vi "RemoteVI Fixture.vi"() -> ()   [LabVIEW 2020]
doc: "Event-logging test fixture of the RemoteVI integration tests (tests\\lv). At start it truncates or creates the log file (Log Path, or RemoteVI Fixture.log in the system temp directory when Log Path is empty), writes one layout line per logged control with its body rectangle in panel-image coordinates, publishes its own front panel with RemoteVI Start.vi on port 8089 and writes ready. An event loop then appends one tab-separated line per handled event - value changes of Switch, Button, Number, Text, Mode and Tab (Tab registered dynamically, because the tab control is pasted in after generation), mouse down and up on Switch, Button, Number and Text, mouse enter and leave on Button, key down on Text and Number, double click on List with the row, mouse wheel on Number with the delta, the selection in the run-time shortcut menu of Text by item tag (the menu is rebuilt in Shortcut Menu Activation? as Top and More with the submenu item Deep), the selection in the VI's run-time menu bar by item tag (built at start: one menu Fixture with Say Hello (tag Hello) and the submenu More with Deep Bar (tag DeepBar)), the answer of the Two Button Dialog Proceed? (Yes / No) that the latched button Ask opens (dialog TRUE or FALSE) and the result of the native File Dialog that the latched button Open opens (file and the path, or CANCELLED) - in the format documented in tests\\lv\\harness.mjs, while a parallel loop redraws a moving sine on Graph every 50 ms and logs scroll x y whenever the panel was scrolled (Front Panel Window:Origin changed); 1.5 s after the last scroll it scrolls the panel back to 0,0, so a later test run finds the controls where the layout lines say. Stop ends both loops, the log is closed and RemoteVI Stop.vi releases the port. error out merges every error path."
uses:
  source/RemoteVI.lvlib
panel:
  in  "Tab":enum32{"One", "Two"}(tab)
  out "error out":errorcluster
  out "Graph":dbl[](graph)
  in  "Stop":bool
  in  "Open":bool
  in  "Ask":bool
  in  "List":i32(listbox)
  in  "Mode":i32(ring) items=["Off", "Slow", "Fast"]
  in  "Text":string
  in  "Number":dbl
  in  "Button":bool
  in  "Switch":bool
  in  "Log Path":path
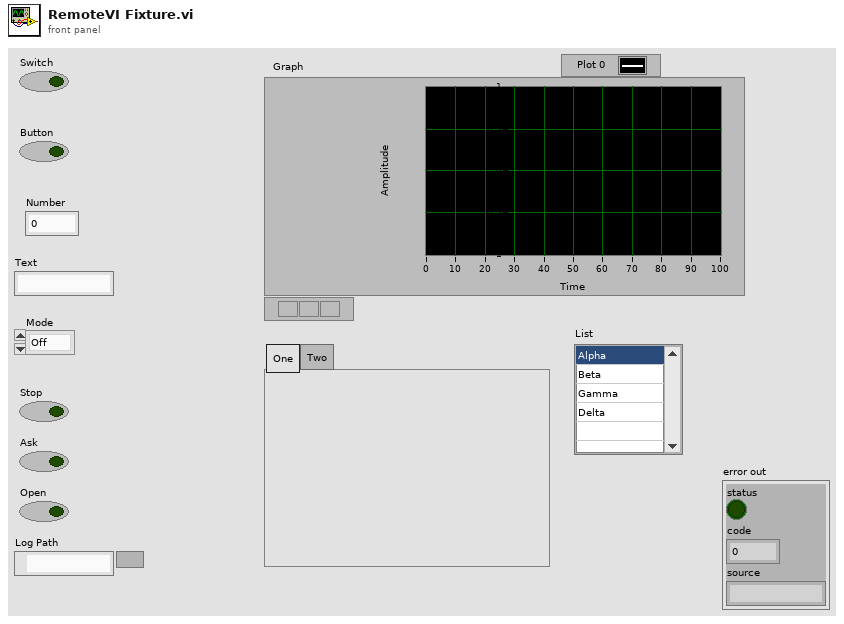
[diagram p1: front panel]
types:
  T1 = enum16{"open", "replace", "create", "open or create", "replace or create", "replace or create with confirmation"}
  T2 = typedef "LVPointTypeDef.ctl" = cluster{"Horizontal":i16, "Vertical":i16}
  T3 = typedef "LVPoint32TypeDef.ctl" = cluster{"Horizontal":i32, "Vertical":i32}
  T4 = cluster{"Shift":bool, "Ctrl":bool, "Alt":bool, "Cmd":bool, "Opt":bool}
  T5 = typedef "eventvkey.ctl" = enum16{"ASCII", "Enter", "Return", "Shift", "Ctrl", "Alt", "Cmd", "Opt", "Caps", "NumLock", "Clear", "Break", "Up", "Down", "Left", "Right", "Insert", "Delete", "Home", "End", "PageUp", "PageDown", "Escape", "Help", "Pause", "ScrollLock", "F1", "F2", "F3", "F4", "F5", "F6", "F7", "F8", "F9", "F10", "F11", "F12", "F13", "F14", "F15", "F16", "F17", "F18", "F19", "F20", "F21", "F22", "F23", "F24", "Play", "VolumeUp", "VolumeDown", "Mute", "Two Byte Char"}
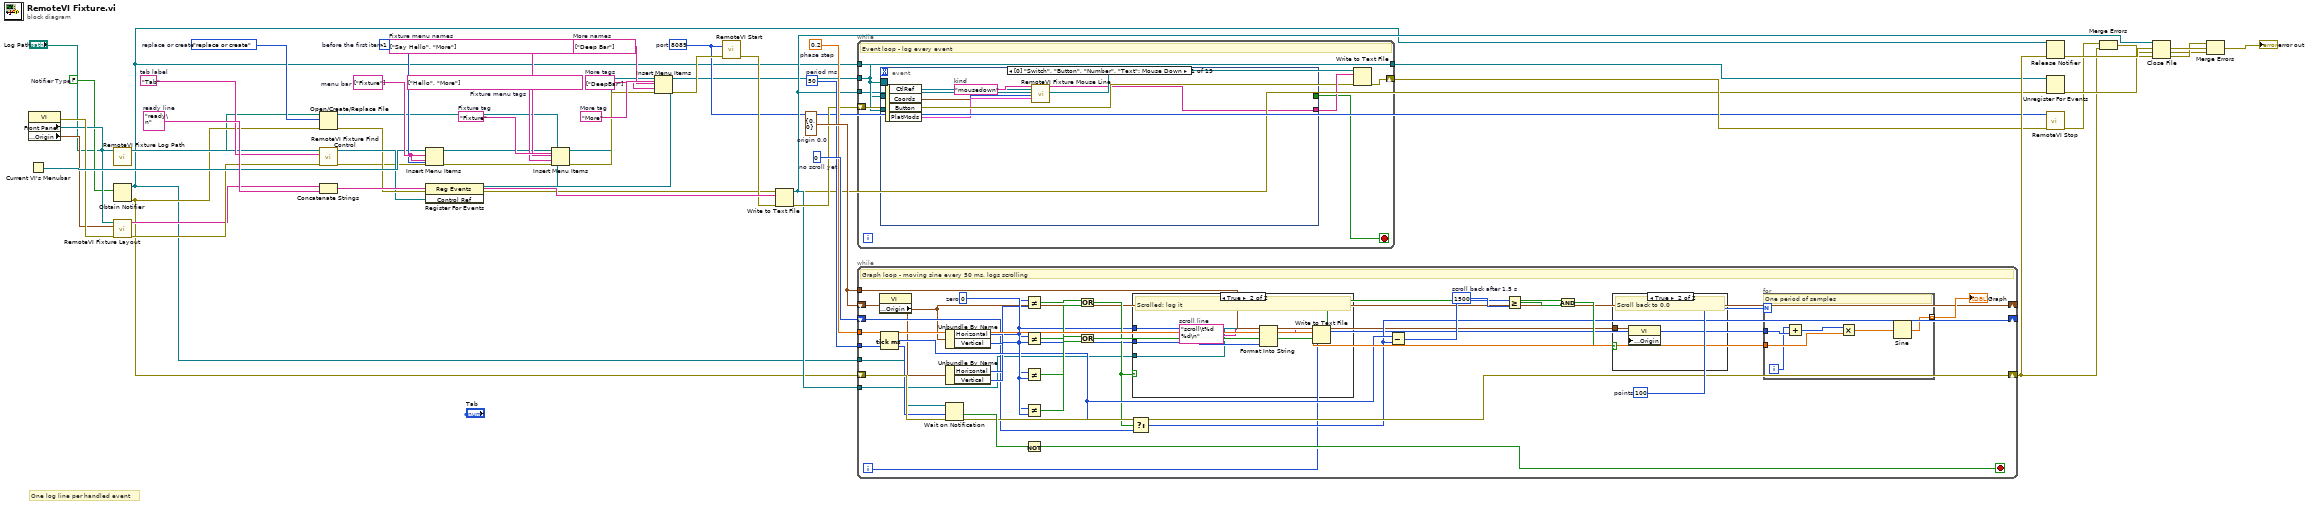
[diagram p0: block diagram]
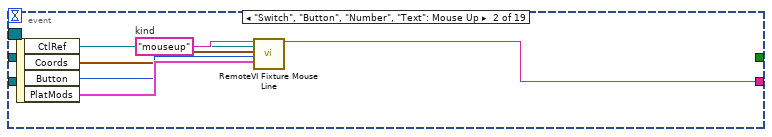
[diagram p4: hidden frame]
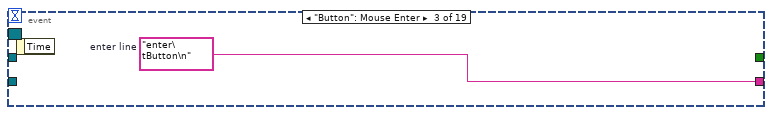
[diagram p5: hidden frame]
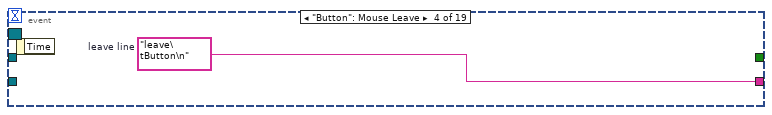
[diagram p6: hidden frame]
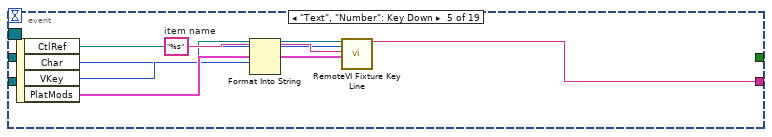
[diagram p7: hidden frame]
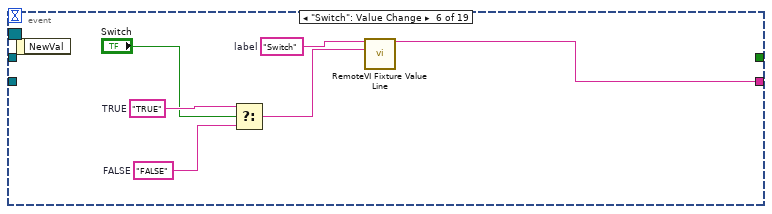
[diagram p8: hidden frame]
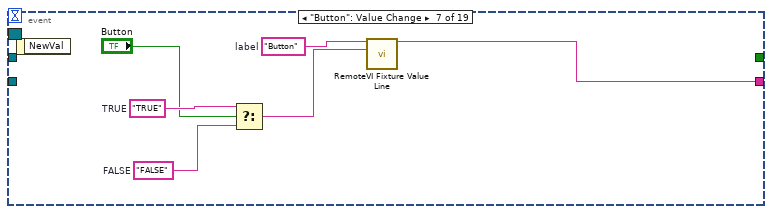
[diagram p9: hidden frame]
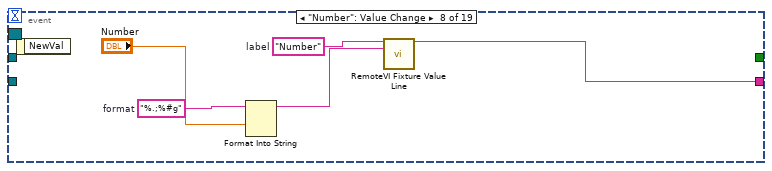
[diagram p10: hidden frame]
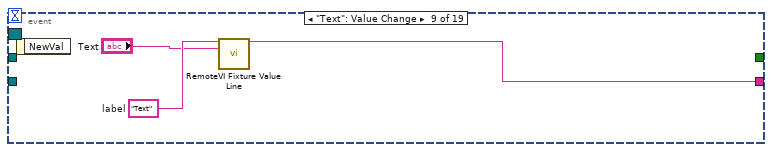
[diagram p11: hidden frame]
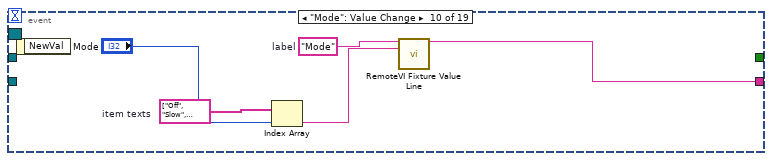
[diagram p12: hidden frame]
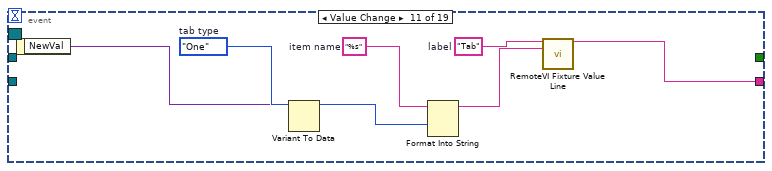
[diagram p13: hidden frame]
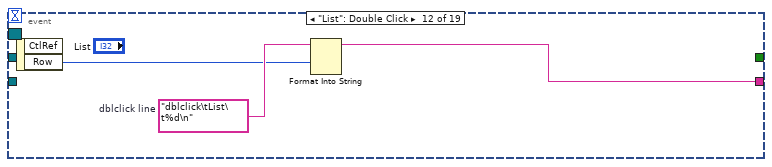
[diagram p14: hidden frame]
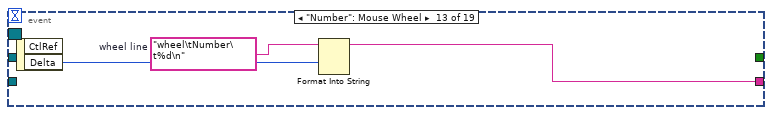
[diagram p15: hidden frame]
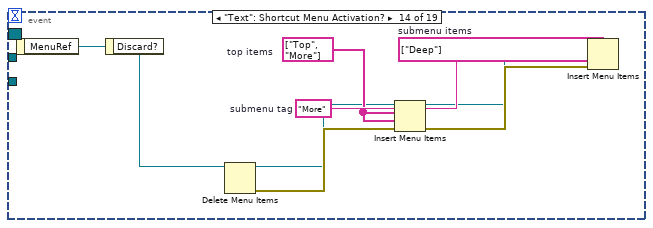
[diagram p16: hidden frame]
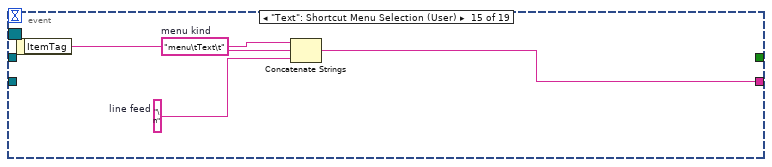
[diagram p17: hidden frame]
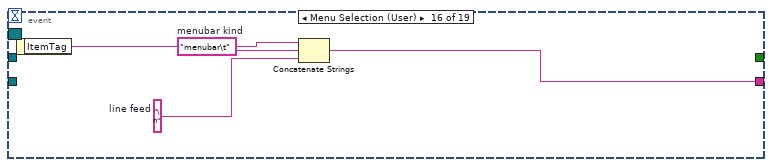
[diagram p18: hidden frame]
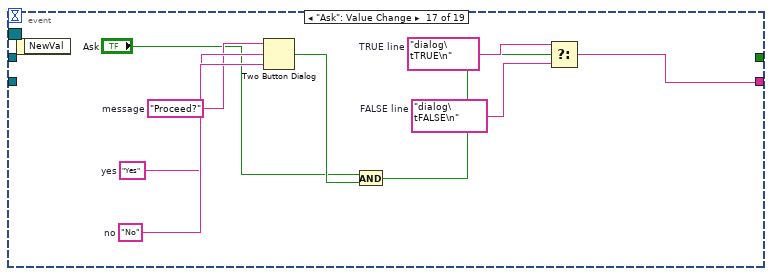
[diagram p19: hidden frame]
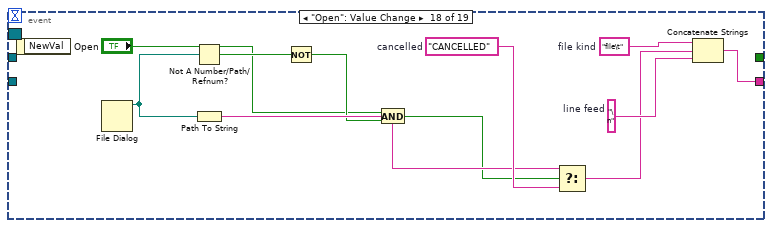
[diagram p20: hidden frame]
diagram:
  w44 = u32 0  # no scroll yet
  w43 = cluster{"Horizontal":i32, "Vertical":i32} {"Horizontal"=0, "Vertical"=0}  # origin 0,0
  w42 = 50  # period ms
  w41 = 0.2  # phase step
  w35 = "ready\n"  # ready line
  w32 = "More"  # More tag
  w31 = string[] ["DeepBar"]  # More tags
  w30 = string[] ["Deep Bar"]  # More names
  w27 = "Fixture"  # Fixture tag
  w26 = string[] ["Hello", "More"]  # Fixture menu tags
  w25 = string[] ["Say Hello", "More"]  # Fixture menu names
  w22 = string[] ["Fixture"]  # menu bar
  w21 = -1  # before the first item
  w19 = u16 8089  # port
  w14 = "Tab"  # tab label
  w6 = T1."replace or create"  # replace or create
  w3 = FALSE  # Notifier Type
  # "One log line per handled event"
  n1 = property class="VI"() -> (error out=w11:errorcluster, "Front Panel"=w9:refnum<vi>, "Front Panel Window:Origin"=w10:T2)  [unwired: 2 in, 1 out]
  n2 = Current VI's Menubar() -> (w20:refnum<k9>)
  n3 = call "RemoteVI Fixture Log Path.vi"("Log Path"="Log Path") -> ("path"=w2:path)  [unwired: 13 in, 1 out]
  n4 = Obtain Notifier(notification data type=w3) -> (notifier out=w4:refnum<notifier>, error out=w5:errorcluster)  [unwired: 3 in, 1 out]
  n5 = call "RemoteVI Fixture Layout.vi"("Panel"=w9, "Origin"=w10, "error in"=w11) -> ("layout"=w12:string, "error out"=w13:errorcluster)  [unwired: 11 in]
  n6 = Open/Create/Replace File(file path (use dialog)=w2, error in=w5, operation (0:open)=w6) -> (refnum out=w7:refnum<file>, error out=w8:errorcluster)  [unwired: 3 in, 1 out]
  n7 = call "RemoteVI Fixture Find Control.vi"("Panel"=w9, "label"=w14, "error in"=w13) -> ("Control Ref"=w15:refnum<vi>, "error out"=w16:errorcluster)  [unwired: 11 in]
  n8 = Concatenate Strings(w12, w35) -> (w36:string)
  n9 = Insert Menu Items(4:w21, 6:w8, 7:w22, 8:w22, 9:w20) -> (0:w24:errorcluster, 3:w23:refnum<k9>)  [unwired: 1 in, 1 out]
  n10 = register-events(error in=w16, w15) -> (reference out=w17:refnum<event-registration>, error out=w18:errorcluster)  [unwired: 1 in]
  n11 = Insert Menu Items(5:w27, 6:w24, 7:w26, 8:w25, 9:w23) -> (0:w29:errorcluster, 3:w28:refnum<k9>)  [unwired: 1 in, 1 out]
  n12 = Insert Menu Items(5:w32, 6:w29, 7:w31, 8:w30, 9:w28) -> (0:w33:errorcluster)  [unwired: 1 in, 2 out]
  n13 = call "RemoteVI Start.vi"("port"=w19, "error in"=w33) -> ("error out"=w34:errorcluster)  [unwired: 12 in, 1 out]
  n14 = Write to Text File(file (use dialog)=w7, text=w36, error in=w34) -> (refnum out=w37:refnum<file>, error out=w38:errorcluster)  [unwired: 1 in, 1 out]
  n15 = while {
    tunnel: w4 -> [w52]
    tunnel: w17 -> [w54]
    tunnel: [w54] -> w40
    tunnel: w37 -> [w53]
    shift-right: [w56] -> w39
    shift-left: w38 -> [w55]
    stop <- w57 stop-if-true
    # "Event loop - log every event"
    n16 = event shown="[0] \"Switch\", \"Button\", \"Number\", \"Text\": Mouse Down" {
      selector: w54 -> [_ _ _ _ _ _ _ _ _ _ _ _ _ _ _ _ _ _ _]
      dyn-events: _ -> [_ _ _ _ _ _ _ _ _ _ _ _ _ _ _ _ _ _ _]
      timeout: _ -> [_ _ _ _ _ _ _ _ _ _ _ _ _ _ _ _ _ _ _]
      tunnel: [_ _ _ _ _ _ _ _ _ _ _ _ _ _ _ _ _ _ "Stop"] -> w57
      tunnel: w52 -> [_ _ _ _ _ _ _ _ _ _ _ _ _ _ _ _ _ _ w154]
      tunnel: [w64 w70 w71 w72 w79 w85 w91 w96 w99 w104 w111 w114 w117 _ w129 w133 w142 w153 _] -> w58
      tunnel: w54 -> [_ _ _ _ _ _ _ _ _ _ _ _ _ _ _ _ _ _ _]
      event "Switch", "Button", "Number", "Text": Mouse Down {
        w63 = "mousedown"  # kind
        n17 = event-data() -> ("CtlRef"=w59:refnum<vi>, "Coords"=w60:T3, "Button"=w61:u16, "PlatMods"=w62:T4)  [unwired: 1 in]
        n18 = call "RemoteVI Fixture Mouse Line.vi"("kind"=w63, "CtlRef"=w59, "Coords"=w60, "Button"=w61, "PlatMods"=w62) -> ("line"=w64:string)  [unwired: 13 in, 1 out]
      }
      event "Switch", "Button", "Number", "Text": Mouse Up {
        w69 = "mouseup"  # kind
        n19 = event-data() -> ("CtlRef"=w65:refnum<vi>, "Coords"=w66:T3, "Button"=w67:u16, "PlatMods"=w68:T4)  [unwired: 1 in]
        n20 = call "RemoteVI Fixture Mouse Line.vi"("kind"=w69, "CtlRef"=w65, "Coords"=w66, "Button"=w67, "PlatMods"=w68) -> ("line"=w70:string)  [unwired: 13 in, 1 out]
      }
      event "Button": Mouse Enter {
        w71 = "enter\tButton\n"  # enter line
        n21 = event-data() -> ()  [unwired: 1 in, 1 out]
      }
      event "Button": Mouse Leave {
        w72 = "leave\tButton\n"  # leave line
        n22 = event-data() -> ()  [unwired: 1 in, 1 out]
      }
      event "Text", "Number": Key Down {
        w77 = "%s"  # item name
        n23 = event-data() -> ("CtlRef"=w73:refnum<vi>, "Char"=w74:i16, "VKey"=w75:T5, "PlatMods"=w76:T4)  [unwired: 1 in]
        n24 = Format Into String(format string=w77, w75) -> (resulting string=w78:string)  [unwired: 2 in, 1 out]
        n25 = call "RemoteVI Fixture Key Line.vi"("CtlRef"=w73, "Char"=w74, "VKey"=w78, "PlatMods"=w76) -> ("line"=w79:string)  [unwired: 14 in, 1 out]
      }
      event "Switch": Value Change {
        w83 = "FALSE"  # FALSE
        w82 = "TRUE"  # TRUE
        w81 = "Switch"  # label
        n26 = event-data() -> ()  [unwired: 1 in, 1 out]
        n27 = Select(t=w82, s="Switch", f=w83) -> (s? t:f=w84:string)
        n28 = call "RemoteVI Fixture Value Line.vi"("label"=w81, "value"=w84) -> ("line"=w85:string)  [unwired: 12 in, 1 out]
      }
      event "Button": Value Change {
        w89 = "FALSE"  # FALSE
        w88 = "TRUE"  # TRUE
        w87 = "Button"  # label
        n29 = event-data() -> ()  [unwired: 1 in, 1 out]
        n30 = Select(t=w88, s="Button", f=w89) -> (s? t:f=w90:string)
        n31 = call "RemoteVI Fixture Value Line.vi"("label"=w87, "value"=w90) -> ("line"=w91:string)  [unwired: 12 in, 1 out]
      }
      event "Number": Value Change {
        w94 = "%.;%#g"  # format
        w93 = "Number"  # label
        n32 = event-data() -> ()  [unwired: 1 in, 1 out]
        n33 = Format Into String(format string=w94, "Number") -> (resulting string=w95:string)  [unwired: 2 in, 1 out]
        n34 = call "RemoteVI Fixture Value Line.vi"("label"=w93, "value"=w95) -> ("line"=w96:string)  [unwired: 12 in, 1 out]
      }
      event "Text": Value Change {
        w98 = "Text"  # label
        n35 = event-data() -> ()  [unwired: 1 in, 1 out]
        n36 = call "RemoteVI Fixture Value Line.vi"("label"=w98, "value"="Text") -> ("line"=w99:string)  [unwired: 12 in, 1 out]
      }
      event "Mode": Value Change {
        w102 = string[] ["Off", "Slow", "Fast"]  # item texts
        w101 = "Mode"  # label
        n37 = event-data() -> ()  [unwired: 1 in, 1 out]
        n38 = Index Array(array=w102, index="Mode") -> (element=w103:string)
        n39 = call "RemoteVI Fixture Value Line.vi"("label"=w101, "value"=w103) -> ("line"=w104:string)  [unwired: 12 in, 1 out]
      }
      event Value Change {
        w109 = "%s"  # item name
        w108 = "Tab"  # label
        w106 = enum32{"One", "Two"}."One"  # tab type
        n40 = event-data() -> ("NewVal"=w105:variant)  [unwired: 1 in]
        n41 = Variant To Data(type=w106, Variant=w105) -> (data=w107:enum32{"One", "Two"})  [unwired: 1 in, 1 out]
        n42 = Format Into String(format string=w109, w107) -> (resulting string=w110:string)  [unwired: 2 in, 1 out]
        n43 = call "RemoteVI Fixture Value Line.vi"("label"=w108, "value"=w110) -> ("line"=w111:string)  [unwired: 12 in, 1 out]
      }
      event "List": Double Click {
        w113 = "dblclick\tList\t%d\n"  # dblclick line
        n44 = event-data() -> ("Row"=w112:i32)  [unwired: 1 in, 1 out]
        n45 = Format Into String(format string=w113, w112) -> (resulting string=w114:string)  [unwired: 2 in, 1 out]
      }
      event "Number": Mouse Wheel {
        w116 = "wheel\tNumber\t%d\n"  # wheel line
        n46 = event-data() -> ("Delta"=w115:i32)  [unwired: 1 in, 1 out]
        n47 = Format Into String(format string=w116, w115) -> (resulting string=w117:string)  [unwired: 2 in, 1 out]
      }
      event "Text": Shortcut Menu Activation? {
        w125 = "More"  # submenu tag
        w124 = string[] ["Deep"]  # submenu items
        w121 = string[] ["Top", "More"]  # top items
        n48 = event-data() -> ("MenuRef"=w118:refnum<k9>)  [unwired: 1 in]
        n49 = event-data() -> ()  [unwired: 2 in, 1 out]
        n50 = Delete Menu Items(9:w118) -> (0:w120:errorcluster, 3:w119:refnum<k9>)  [unwired: 3 in]
        n51 = Insert Menu Items(6:w120, 7:w121, 8:w121, 9:w119) -> (0:w123:errorcluster, 3:w122:refnum<k9>)  [unwired: 2 in, 1 out]
        n52 = Insert Menu Items(5:w125, 6:w123, 7:w124, 8:w124, 9:w122) -> ()  [unwired: 1 in, 3 out]
      }
      event "Text": Shortcut Menu Selection (User) {
        w128 = "\n"  # line feed
        w127 = "menu\tText\t"  # menu kind
        n53 = event-data() -> ("ItemTag"=w126:string)  [unwired: 1 in]
        n54 = Concatenate Strings(w127, w126, w128) -> (w129:string)
      }
      event Menu Selection (User) {
        w132 = "\n"  # line feed
        w131 = "menubar\t"  # menubar kind
        n55 = event-data() -> ("ItemTag"=w130:string)  [unwired: 1 in]
        n56 = Concatenate Strings(w131, w130, w132) -> (w133:string)
      }
      event "Ask": Value Change {
        w141 = "dialog\tFALSE\n"  # FALSE line
        w140 = "dialog\tTRUE\n"  # TRUE line
        w137 = "No"  # no
        w136 = "Yes"  # yes
        w135 = "Proceed?"  # message
        n57 = event-data() -> ()  [unwired: 1 in, 1 out]
        n58 = Two Button Dialog(message=w135, 1:w137, 2:w136) -> (T button?=w138:bool)
        n59 = And(x="Ask", y=w138) -> (x .and. y?=w139:bool)
        n60 = Select(t=w140, s=w139, f=w141) -> (s? t:f=w142:string)
      }
      event "Open": Value Change {
        w152 = "\n"  # line feed
        w151 = "file\t"  # file kind
        w149 = "CANCELLED"  # cancelled
        n61 = event-data() -> ()  [unwired: 1 in, 1 out]
        n62 = File Dialog() -> (3:w144:path)  [unwired: 7 in, 3 out]
        n63 = Not A Number/Path/Refnum?(number/path/refnum=w144) -> (NaN/Path/Refnum?=w145:bool)
        n64 = Path To String(path=w144) -> (string=w148:string)
        n65 = Not(x=w145) -> (.not. x?=w146:bool)
        n66 = And(x="Open", y=w146) -> (x .and. y?=w147:bool)
        n67 = Select(t=w148, s=w147, f=w149) -> (s? t:f=w150:string)
        n68 = Concatenate Strings(w151, w150, w152) -> (w153:string)
      }
      event "Stop": Value Change {
        n69 = event-data() -> ()  [unwired: 1 in, 1 out]
        n70 = Send Notification(notification="Stop", notifier=w154) -> ()  [unwired: 1 in, 2 out]
      }
    }
    n71 = Write to Text File(file (use dialog)=w53, text=w58, error in=w55) -> (error out=w56:errorcluster)  [unwired: 1 in, 2 out]
  }
  n72 = while {
    tunnel: w43 -> [w159]
    shift-right: [w161] -> _
    shift-left: w43 -> [w160]
    shift-right: [w163] -> _
    shift-left: w44 -> [w162]
    tunnel: w41 -> [w180]
    tunnel: w42 -> [w181]
    tunnel: w4 -> [w157]
    shift-right: [w183] -> w45
    shift-left: w5 -> [w182]
    tunnel: w37 -> [w158]
    i -> [w156]
    stop <- w187 stop-if-true
    w185 = 100  # points
    w177 = u32 1500  # scroll back after 1.5 s
    w172 = 0  # zero
    # "Graph loop - moving sine every 50 ms, logs scrolling"
    n73 = property class="VI"() -> ("Front Panel Window:Origin"=w161:T2)  [unwired: 2 in, 2 out]
    n74 = Tick Count (ms)() -> (millisecond timer value=w171:u32)
    n75 = Unbundle By Name(w161) -> ("Horizontal"=w164:i16, "Vertical"=w165:i16)
    n76 = Unbundle By Name(w160) -> ("Horizontal"=w166:i32, "Vertical"=w167:i32)
    n77 = Wait on Notification(notifier=w157, timeout in ms (-1)=w181, error in (no error)=w182) -> (timed out?=w184:bool, error out=w183:errorcluster)  [unwired: 1 in, 2 out]
    n78 = Not Equal?(x=w164, y=w166) -> (x != y?=w168:bool)
    n79 = Not Equal?(x=w165, y=w167) -> (x != y?=w169:bool)
    n80 = Not Equal?(x=w164, y=w172) -> (x != y?=w173:bool)
    n81 = Not Equal?(x=w165, y=w172) -> (x != y?=w174:bool)
    n82 = Not(x=w184) -> (.not. x?=w187:bool)
    n83 = Or(x=w168, y=w169) -> (x .or. y?=w170:bool)
    n84 = Or(x=w173, y=w174) -> (x .or. y?=w175:bool)
    n85 = case shown="True" w170 {
      tunnel: w164 -> [_ w196]
      tunnel: w165 -> [_ w197]
      tunnel: w158 -> [_ w195]
      frame False {
      }
      frame True {
        w198 = "scroll\t%d %d\n"  # scroll line
        # "Scrolled: log it"
        n86 = Format Into String(format string=w198, w196, w197) -> (resulting string=w199:string)  [unwired: 2 in, 1 out]
        n87 = Write to Text File(file (use dialog)=w195, text=w199) -> ()  [unwired: 2 in, 3 out]
      }
    }
    n88 = Select(t=w171, s=w170, f=w162) -> (s? t:f=w163:u32)
    n89 = Subtract(x=w171, y=w163) -> (x-y=w176:u32)
    n90 = Greater Or Equal?(x=w176, y=w177) -> (x >= y?=w178:bool)
    n91 = And(x=w175, y=w178) -> (x .and. y?=w179:bool)
    n92 = case shown="True" w179 {
      tunnel: w159 -> [_ w194]
      frame False {
      }
      frame True {
        # "Scroll back to 0,0"
        n93 = property class="VI"("Front Panel Window:Origin"=w194) -> ()  [unwired: 2 in, 2 out]
      }
    }
    n94 = for {
      N: w185 -> [_]
      tunnel: w156 -> [w189]
      tunnel: w180 -> [w190]
      tunnel: [w193] -> w186 mode=indexing
      i -> [w188]
      # "One period of samples"
      n95 = Add(x=w188, y=w189) -> (x+y=w191:i32)
      n96 = Multiply(x=w191, y=w190) -> (x*y=w192:dbl)
      n97 = Sine(x=w192) -> (sin(x)=w193:dbl)
    }
    "Graph" <- w186
  }
  n98 = Release Notifier(notifier=w4, error in (no error)=w45) -> (error out=w50:errorcluster)  [unwired: 1 in, 2 out]
  n99 = Unregister For Events(event registration refnum=w40, error in=w18) -> (error out=w47:errorcluster)
  n100 = call "RemoteVI Stop.vi"("port"=w19, "error in"=w39) -> ("error out"=w46:errorcluster)  [unwired: 13 in]
  n101 = Merge Errors(w46, w45) -> (w48:errorcluster)
  n102 = Close File(refnum=w37, error in=w48) -> (error out=w49:errorcluster)  [unwired: 1 out]
  n103 = Merge Errors(w49, w50, w47) -> (→"error out":errorcluster)
